vi "Unpack.vi"(8 "error in":errorcluster, 10 "destination folder":path, 11 "nipkg filepath":path) -> (0 "error out":errorcluster, 1 "instructions filepath":path, 2 "control filepath":path, 3 "unpacked folderpath":path, 5 "data folderpath":path)   [LabVIEW 2014, in "NIPM_API.lvlib"]
doc: "Unpacks an existing package file (.nipkg) to a nipkg folder structure\n\nINPUT(s)\n<B>nipkg filepath</B>: Specifies the filepath of the package (.nipkg) to unpack\n\n<B>Destination folder</B>: Specifies the destination folder in which this VI will output the unpacked nipkg folder structure\n\nOUTPUT(s)\n<B>Unpacked folderpath</B>: Outputs the path of the folder containing the unpacked nipkg folder structure that this VI created\n\n<B>Control filepath</B>: Outputs the control filepath in the unpacked nipkg folder structure\n\n<B>Instructions filepath</B>: Outputs instructions filepath in the unpacked nipkg folder structure\n\n<B>Data folderpath</B>: Outputs the data folderpath in the unpacked nipkg folder structure\n\nDETAILS\nFor additional details on the nipkg folder structure, refer to the following link:\nhttp://www.ni.com/documentation/en/ni-package-manager/latest/manual/assemble-file-package/"
uses:
  NIPM_API.lvlib
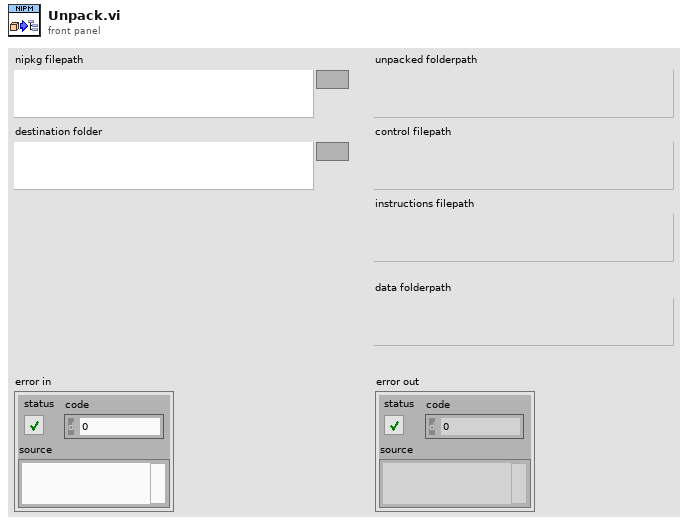
[diagram p1: front panel]
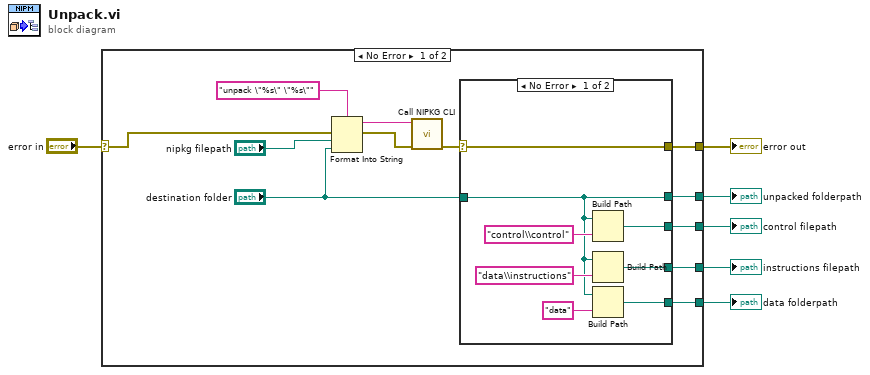
[diagram p0: block diagram]
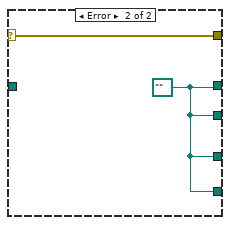
[diagram p2: hidden frame]
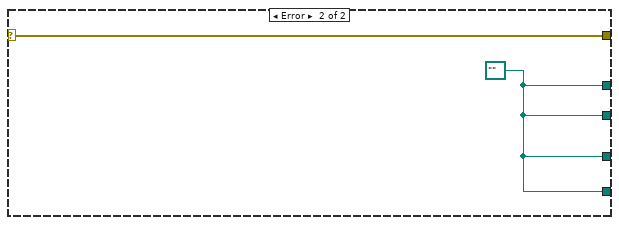
[diagram p3: hidden frame]
diagram:
  n1 = case shown="No Error" "error in" {
    selector: "error in" -> [w16 w30]
    tunnel: [w12 w30] -> w5
    tunnel: [w10 w29] -> w4
    tunnel: [w9 w29] -> w3
    tunnel: [w8 w29] -> w2
    tunnel: [w7 w29] -> w1
    frame No Error {
      n2 = Format Into String(format string="unpack \"%s\" \"%s\"", error in=w16, "nipkg filepath", "destination folder") -> (resulting string=w15:string, error out=w14:errorcluster)  [unwired: 1 in]
      n3 = call "Call NIPKG CLI.vi"("error in (no error)"=w14, "command"=w15) -> ("error out"=w13:errorcluster)  [unwired: 8 in, 1 out]
      n4 = case shown="No Error" w13 {
        selector: w13 -> [w26 w28]
        tunnel: [w26 w28] -> w12
        tunnel: [w19 w27] -> w10
        tunnel: "destination folder" -> [w19 _]
        tunnel: [w24 w27] -> w9
        tunnel: [w22 w27] -> w8
        tunnel: [w20 w27] -> w7
        frame No Error {
          n5 = Build Path(base path=w19, name or relative path="control\\control") -> (appended path=w24:path)
          n6 = Build Path(base path=w19, name or relative path="data\\instructions") -> (appended path=w22:path)
          n7 = Build Path(base path=w19, name or relative path="data") -> (appended path=w20:path)
        }
        frame Error {
          w27 = path "" ("t")
        }
      }
    }
    frame Error {
      w29 = path "" ("destination folder")
    }
  }
  "error out" <- w5
  "unpacked folderpath" <- w4
  "control filepath" <- w3
  "instructions filepath" <- w2
  "data folderpath" <- w1
